vi "AO Python Get Image.vi"(0 "Camera Notifier":string, 2 "Use ROI":bool) -> (8 "Image Out":dbl[][][](array[numeric]), 13 "2D Image":u16[][](array[numeric]))   [LabVIEW 2016]
uses:
  Device Library/Cameras/Camera Controls/Camera IMAQ Key Info.ctl
  Device Library/Cameras/Photometrics/Prime BSI/Prime BSI Controls/Prime Actions.ctl
  Device Library/Cameras/Hamamatsu/Orca Flash/Orca Flash Controls/Orca Flash Actions.ctl
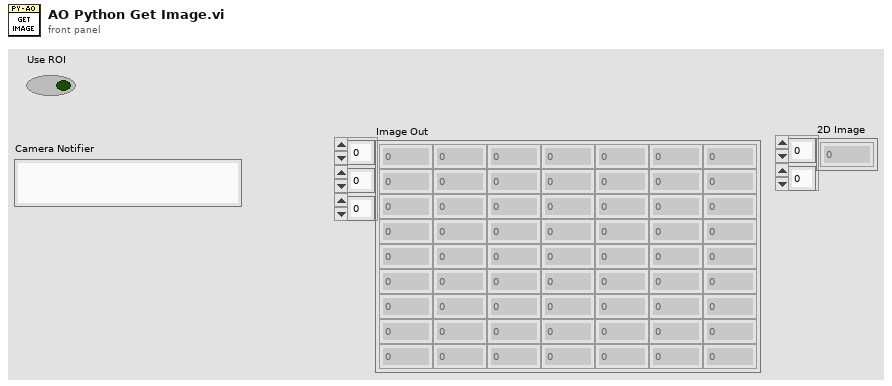
[diagram p1: front panel]
types:
  T1 = typedef "Camera IMAQ Key Info.ctl" = cluster{"Frame":u32, "Sensor Height":i32, "Sensor Width":i32, "ROI Height":i32, "ROI Width":i32, "ROI Enable?":bool, "Bit per Pixel":u8}
  T2 = typedef "Orca Flash Actions.ctl" = enum16{"IDLE", "PREVIEW", "RECORD", "Record Settings", "SETPARAM", "GETPARAM", "SETROI", "GETROI", "PROGRESSIVE MODE", "AREA MODE", "STATUS", "QUIT"}
  T3 = typedef "Prime Actions.ctl" = enum16{"Error Check", "Initialize", "Preview", "Record", "Abort", "Record Settings", "Set Parameter", "Get Parameter", "Set ROI", "Get ROI", "Status", "Set Trigger", "Quit"}
  T4 = typedef "IMAQ Image.ctl" = refnum<image>
  T5 = typedef "Image Type" = u32
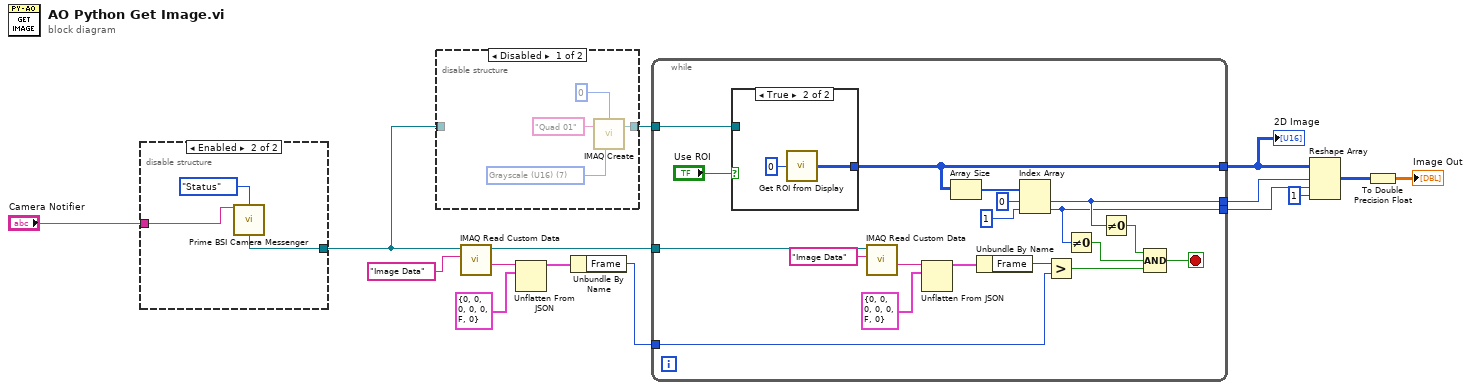
[diagram p0: block diagram]
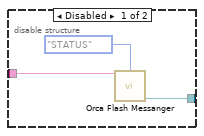
[diagram p3: hidden frame]
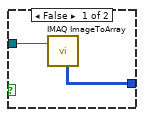
[diagram p4: hidden frame]
diagram:
  n1 = disable-structure shown="Enabled" {
    disable-tunnel: "Camera Notifier" -> [w18 w20]
    disable-tunnel: [w16 w21] -> w1
    frame Disabled {
      n2 = call "Orca Flash Messanger.vi"("Notifier Name"=w18, "Camera Actions"=Orca_Flash_Actions."STATUS") -> ("Image Ref"=w16:T4)  [unwired: 9 in, 4 out]
    }
    frame Enabled {
      n3 = call "Prime BSI Camera Messenger.vi"("Notifier Name"=w20, "Prime Actions"=Prime_Actions."Status") -> ("Image Ref"=w21:T4)  [unwired: 8 in, 5 out]
    }
  }
  n4 = disable-structure shown="Disabled" {
    disable-tunnel: [w22 w26] -> w2
    disable-tunnel: w1 -> [_ w26]
    frame Disabled {
      w23 = T5 7 items=["Grayscale (U8)", "Grayscale (I16)", "Grayscale (SGL)", "Complex (CSG)", "RGB (U32)", "HSL (U32)", "RGB (U64)", "Grayscale (U16)"] ("Image Type")
      n5 = call "IMAQ Create"("Border Size"=0, "Image Name"="Quad 01", "Image Type"=w23) -> ("New Image"=w22:T4)  [unwired: 2 in, 1 out]
    }
    frame Enabled {
    }
  }
  n6 = call "IMAQ Read Custom Data"("Key"="Image Data", "Image"=w1) -> ("Custom Data Out"=w13:string, "Image (duplicate)"=w10:T4)  [unwired: 7 in, 1 out]
  n7 = Unflatten From JSON(JSON string=w13, type and defaults=T1 {"Frame"=0, "Sensor Height"=0, "Sensor Width"=0, "ROI Height"=0, "ROI Width"=0, "ROI Enable?"=FALSE, "Bit per Pixel"=0} ("Camera IMAQ Key Info")) -> (value=w11:T1)  [unwired: 5 in, 1 out]
  n8 = Unbundle By Name(w11) -> ("Frame"=w9:u32)
  n9 = while {
    tunnel: w10 -> [w41]
    tunnel: w9 -> [w39]
    tunnel: [w28] -> w6
    tunnel: [w33] -> w4
    tunnel: [w31] -> w5
    tunnel: w2 -> [w29]
    stop <- w34 stop-if-true
    n10 = case shown="True" "Use ROI" {
      tunnel: w29 -> [w47 _]
      tunnel: [w46 w48] -> w28
      frame False {
        n11 = call "IMAQ ImageToArray"("Image"=w47) -> ("Image Pixels (U16)"=w46:u16[][])  [unwired: 3 in, 4 out]
      }
      frame True {
        n12 = call "Get ROI from Display.vi"("Display Index"=0) -> ("Image Out"=w48:u16[][])  [unwired: 14 in]
      }
    }
    n13 = call "IMAQ Read Custom Data"("Key"="Image Data", "Image"=w41) -> ("Custom Data Out"=w44:string)  [unwired: 7 in, 2 out]
    n14 = Unflatten From JSON(JSON string=w44, type and defaults=T1 {"Frame"=0, "Sensor Height"=0, "Sensor Width"=0, "ROI Height"=0, "ROI Width"=0, "ROI Enable?"=FALSE, "Bit per Pixel"=0} ("Camera IMAQ Key Info")) -> (value=w42:T1)  [unwired: 5 in, 1 out]
    n15 = Array Size(array=w28) -> (size(s)=w38:i32[])
    n16 = Unbundle By Name(w42) -> ("Frame"=w40:u32)
    n17 = Index Array(array=w38, index #1=0 ("index"), index #2=1 ("index")) -> (element #1=w33:i32, element #2=w31:i32)
    n18 = Greater?(x=w40, y=w39) -> (0:w35:bool)
    n19 = Not Equal To 0?(x=w31) -> (x != 0?=w30:bool)
    n20 = Not Equal To 0?(x=w33) -> (x != 0?=w32:bool)
    n21 = Compound Arithmetic op=AND(w32, w30, w35) -> (w34:bool)
  }
  "2D Image" <- w6
  n22 = Reshape Array(w6, w4, w5, 1 ("dimension size")) -> (w3:u16[][][])
  n23 = To Double Precision Float(number=w3) -> (double precision float=→"Image Out":dbl[][][])
